vi "subvi.vi"(8 "error in":errorcluster) -> (0 "error out":errorcluster, 3 "Runner's Data Ind":T1)   [LabVIEW 2025]
uses:
  Lab 3/Control Runners.ctl
panel:
  in  "Runner's Data Ctrl":T1
  in  "OK":bool
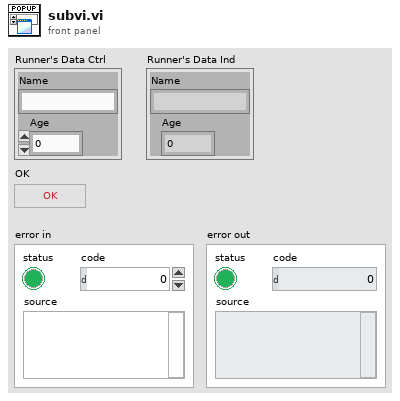
[diagram p1: front panel]
types:
  T1 = typedef "Control Runners.ctl" = cluster{"Name":string, "Age":i32}
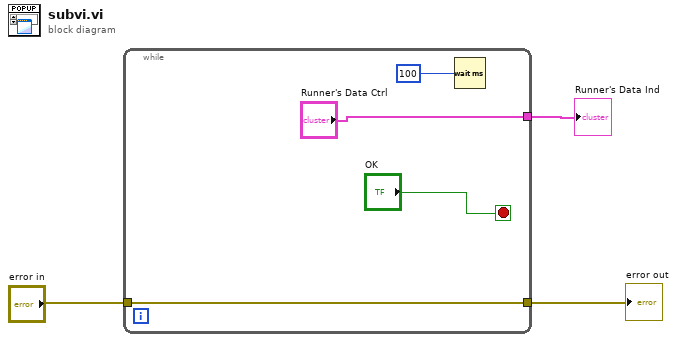
[diagram p0: block diagram]
diagram:
  n1 = while {
    tunnel: ["Runner's Data Ctrl"] -> w3
    tunnel: [w5] -> w2
    tunnel: "error in" -> [w5]
    stop <- "OK" stop-if-true
    n2 = Wait (ms)(milliseconds to wait=u32 100 ("millisecond timer value")) -> ()  [unwired: 1 out]
  }
  "error out" <- w2
  "Runner's Data Ind" <- w3
